vi "Build Shared Library Search Path.vi"(8 "Error In":errorcluster, 11 "LabPack Shared Library":path=path "") -> (0 "Error Out":errorcluster, 3 "Search Path":path[](array[path]))   [LabVIEW 2018, in "Toolkit.lvlib"]
doc: "Builds an array of paths to search for the LabPack shared library based on the target system. This also handles 32-bit and 64-bit systems. On Windows, the shared library is a Dynamic Link Library (DLL). On macOS, the shared library is a Dynamic Library (dylib). On Linux, the shared library is a Shared Object (SO). On Linux RT, the shared library is a Shared Object (SO) but it has a \"-rt\" suffix to the name before the extension."
uses:
  Toolkit.lvlib
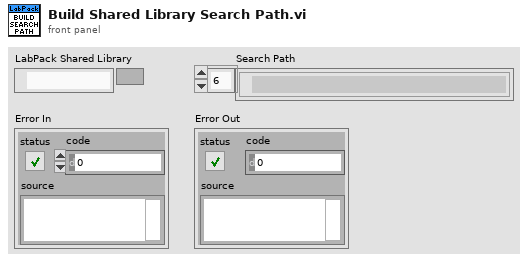
[diagram p1: front panel]
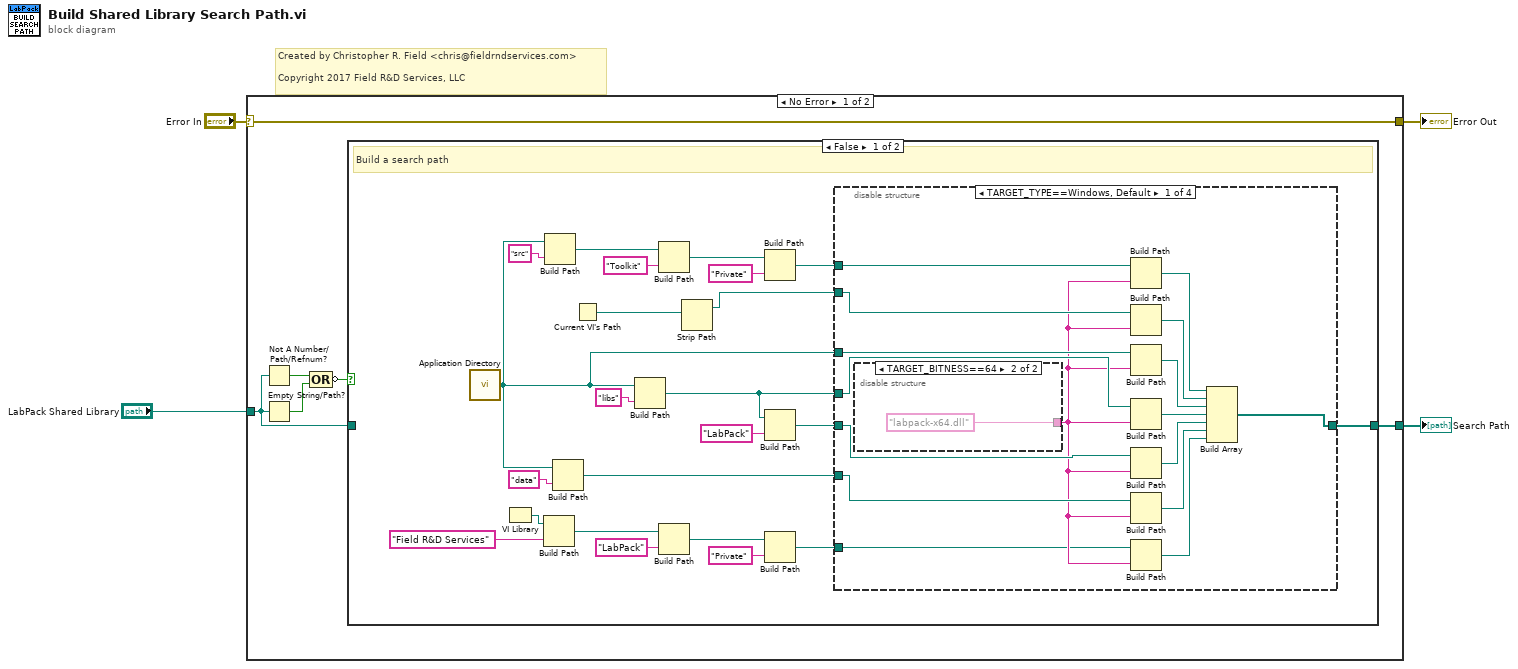
[diagram p0: block diagram]
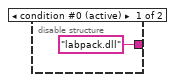
[diagram p2: hidden frame]
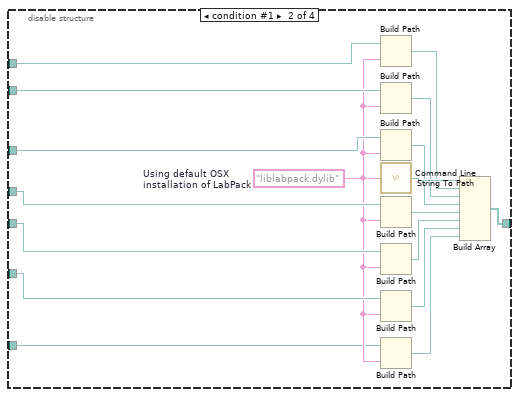
[diagram p3: hidden frame]
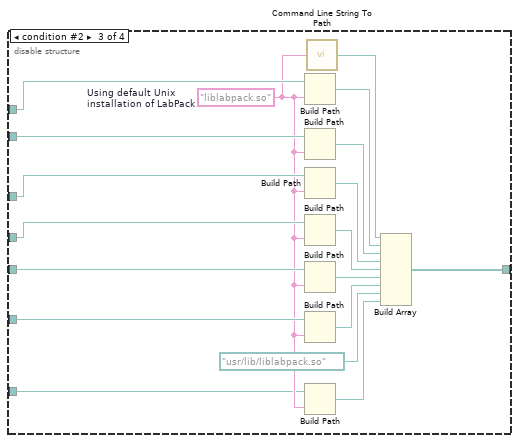
[diagram p4: hidden frame]
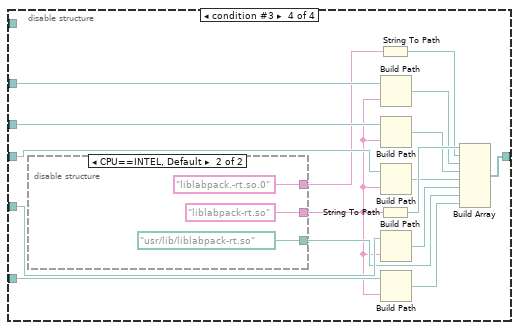
[diagram p5: hidden frame]
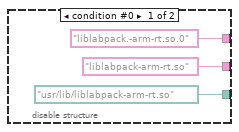
[diagram p6: hidden frame]
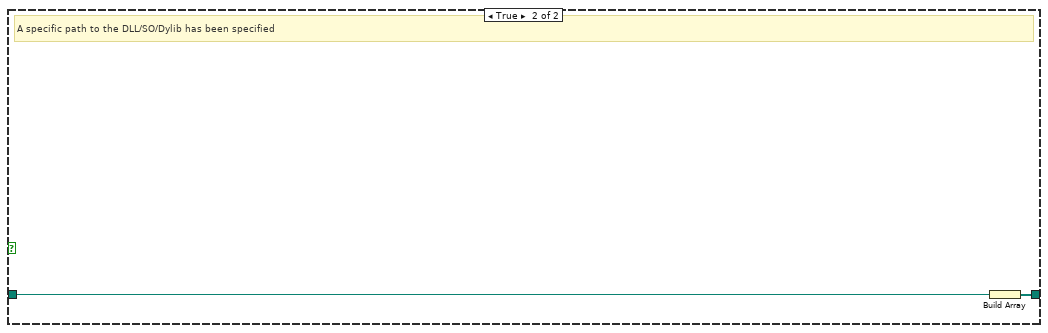
[diagram p7: hidden frame]
diagram:
  # "Created by Christopher R. Field <chris@fieldrndservices.com>\n\nCopyright 2017 Field R&D Services, LLC"
  n1 = case shown="No Error" "Error In" {
    selector: "Error In" -> [w9 w111]
    tunnel: [w10 _] -> w4
    tunnel: "LabPack Shared Library" -> [w6 _]
    tunnel: [w9 w111] -> w1
    frame No Error {
      n2 = Not A Number/Path/Refnum?(number/path/refnum=w6) -> (NaN/Path/Refnum?=w7:bool)
      n3 = Empty String/Path?(string/path=w6) -> (empty?=w8:bool)
      n4 = Compound Arithmetic op=OR(w7, w8) -> (invert w5:bool)
      n5 = case shown="False" w5 {
        tunnel: w6 -> [_ w110]
        tunnel: [w27 w109] -> w10
        frame False {
          # "Build a search path"
          n6 = call <vilib>:"Application Directory.vi"() -> ("Application Directory"=w25:path)
          n7 = VI Library() -> (path=w19:path)
          n8 = Build Path(base path=w19, name or relative path="Field R&D Services") -> (appended path=w17:path)
          n9 = Build Path ("EXE include\nlocation")(base path=w25, name or relative path="src") -> (appended path=w30:path)
          n10 = Build Path ("EXE include\nlocation")(base path=w25, name or relative path="data") -> (appended path=w23:path)
          n11 = Current VI's Path() -> (path=w12:path)
          n12 = Build Path ("EXE include\nlocation")(base path=w25, name or relative path="libs") -> (appended path=w22:path)
          n13 = Build Path ("EXE include\nlocation")(base path=w30, name or relative path="Toolkit") -> (appended path=w32:path)
          n14 = Build Path(base path=w17, name or relative path="LabPack") -> (appended path=w15:path)
          n15 = Strip Path(path=w12) -> (stripped path=w11:path)  [unwired: 1 out]
          n16 = Build Path ("EXE include\nlocation")(base path=w32, name or relative path="Private") -> (appended path=w28:path)
          n17 = Build Path ("EXE include\nlocation")(base path=w22, name or relative path="LabPack") -> (appended path=w20:path)
          n18 = Build Path(base path=w15, name or relative path="Private") -> (appended path=w13:path)
          n19 = disable-structure shown="TARGET_TYPE==Windows, Default" {
            disable-tunnel: [w46 w67 w85 w102] -> w27
            disable-tunnel: w28 -> [w49 w66 w84 _]
            disable-tunnel: w11 -> [w48 w64 w82 _]
            disable-tunnel: w25 -> [w44 w62 w75 w95]
            disable-tunnel: w22 -> [w42 w61 w74 w94]
            disable-tunnel: w23 -> [w41 w59 w72 w92]
            disable-tunnel: w20 -> [w38 w60 w73 w93]
            disable-tunnel: w13 -> [w35 w53 w70 w89]
            frame condition #0 (active) {
              n20 = disable-structure shown="TARGET_BITNESS==64" {
                disable-tunnel: ["labpack.dll" ("name or relative path") "labpack-x64.dll" ("name or relative path")] -> w36
                frame condition #0 (active) {
                }
                frame condition #1 {
                }
              }
              n21 = Build Path ("EXE include\nlocation")(base path=w49, name or relative path=w36) -> (appended path=w47:path)
              n22 = Build Path ("EXE include\nlocation")(base path=w48, name or relative path=w36) -> (appended path=w45:path)
              n23 = Build Path ("EXE include\nlocation")(base path=w44, name or relative path=w36) -> (appended path=w43:path)
              n24 = Build Path ("EXE include\nlocation")(base path=w42, name or relative path=w36) -> (appended path=w40:path)
              n25 = Build Path ("EXE include\nlocation")(base path=w38, name or relative path=w36) -> (appended path=w37:path)
              n26 = Build Path ("EXE include\nlocation")(base path=w41, name or relative path=w36) -> (appended path=w39:path)
              n27 = Build Path ("EXE include\nlocation")(base path=w35, name or relative path=w36) -> (appended path=w34:path)
              n28 = Build Array(w47, w45, w43, w40, w37, w39, w34) -> (w46:path[])
            }
            frame condition #1 {
              w54 = "liblabpack.dylib"  # Using default OSX installation of LabPack
              n29 = Build Path ("EXE include\nlocation")(base path=w66, name or relative path=w54) -> (appended path=w65:path)
              n30 = Build Path ("EXE include\nlocation")(base path=w64, name or relative path=w54) -> (appended path=w63:path)
              n31 = Build Path ("EXE include\nlocation")(base path=w62, name or relative path=w54) -> (appended path=w58:path)
              n32 = call <vilib>:"Command Line String To Path.vi"("string"=w54) -> ("path"=w68:path)
              n33 = Build Path ("EXE include\nlocation")(base path=w61, name or relative path=w54) -> (appended path=w57:path)
              n34 = Build Path ("EXE include\nlocation")(base path=w60, name or relative path=w54) -> (appended path=w56:path)
              n35 = Build Path ("EXE include\nlocation")(base path=w59, name or relative path=w54) -> (appended path=w55:path)
              n36 = Build Path ("EXE include\nlocation")(base path=w53, name or relative path=w54) -> (appended path=w52:path)
              n37 = Build Array(w68, w65, w63, w58, w57, w56, w55, w52) -> (w67:path[])
            }
            frame condition #2 {
              w71 = "liblabpack.so"  # Using default Unix installation of LabPack
              n38 = Build Path ("EXE include\nlocation")(base path=w84, name or relative path=w71) -> (appended path=w83:path)
              n39 = Build Path ("EXE include\nlocation")(base path=w82, name or relative path=w71) -> (appended path=w81:path)
              n40 = Build Path ("EXE include\nlocation")(base path=w75, name or relative path=w71) -> (appended path=w79:path)
              n41 = Build Path ("EXE include\nlocation")(base path=w74, name or relative path=w71) -> (appended path=w78:path)
              n42 = Build Path ("EXE include\nlocation")(base path=w73, name or relative path=w71) -> (appended path=w77:path)
              n43 = Build Path ("EXE include\nlocation")(base path=w72, name or relative path=w71) -> (appended path=w76:path)
              n44 = Build Path ("EXE include\nlocation")(base path=w70, name or relative path=w71) -> (appended path=w69:path)
              n45 = call <vilib>:"Command Line String To Path.vi"("string"=w71) -> ("path"=w86:path)
              n46 = Build Array(w86, w83, w81, w79, w78, w77, w76, path "/usr/lib/liblabpack.so" ("path"), w69) -> (w85:path[])
            }
            frame condition #3 {
              n47 = disable-structure shown="CPU==INTEL, Default" {
                disable-tunnel: ["liblabpack.-arm-rt.so.0" "liblabpack.-rt.so.0"] -> w91
                disable-tunnel: ["liblabpack-arm-rt.so" "liblabpack-rt.so"] -> w88
                disable-tunnel: [path "/usr/lib/liblabpack-arm-rt.so" ("path") path "/usr/lib/liblabpack-rt.so" ("path")] -> w90
                frame condition #0 {
                }
                frame condition #1 (active) {
                }
              }
              n48 = String To Path(string=w91) -> (path=w100:path)
              n49 = String To Path(string=w88) -> (path=w101:path)
              n50 = Build Path ("EXE include\nlocation")(base path=w95, name or relative path=w88) -> (appended path=w96:path)
              n51 = Build Path ("EXE include\nlocation")(base path=w94, name or relative path=w88) -> (appended path=w99:path)
              n52 = Build Path ("EXE include\nlocation")(base path=w93, name or relative path=w88) -> (appended path=w98:path)
              n53 = Build Path ("EXE include\nlocation")(base path=w92, name or relative path=w88) -> (appended path=w97:path)
              n54 = Build Path ("EXE include\nlocation")(base path=w89, name or relative path=w88) -> (appended path=w87:path)
              n55 = Build Array(w101, w100, w96, w99, w98, w97, w90, w87) -> (w102:path[])
            }
          }
        }
        frame True {
          # "A specific path to the DLL/SO/Dylib has been specified"
          n56 = Build Array(w110) -> (w109:path[])
        }
      }
    }
    frame Error {
    }
  }
  "Search Path" <- w4
  "Error Out" <- w1
